vi "Post-Install Custom Action.vi"(10 "Variant":variant) -> (0 "error out":errorcluster)   [LabVIEW 2021]
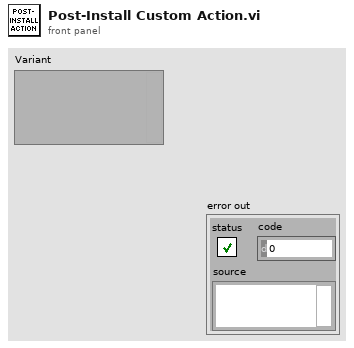
[diagram p1: front panel]
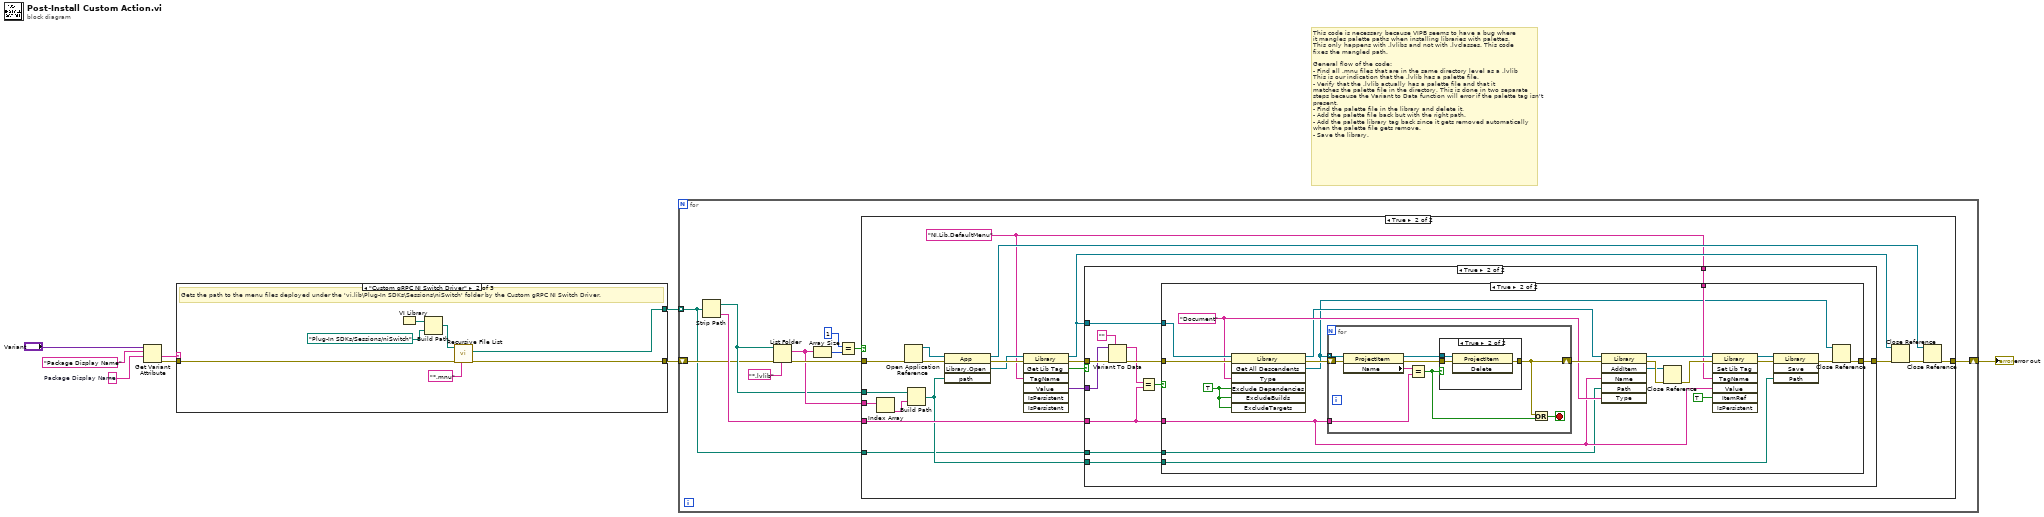
[diagram p0: block diagram]
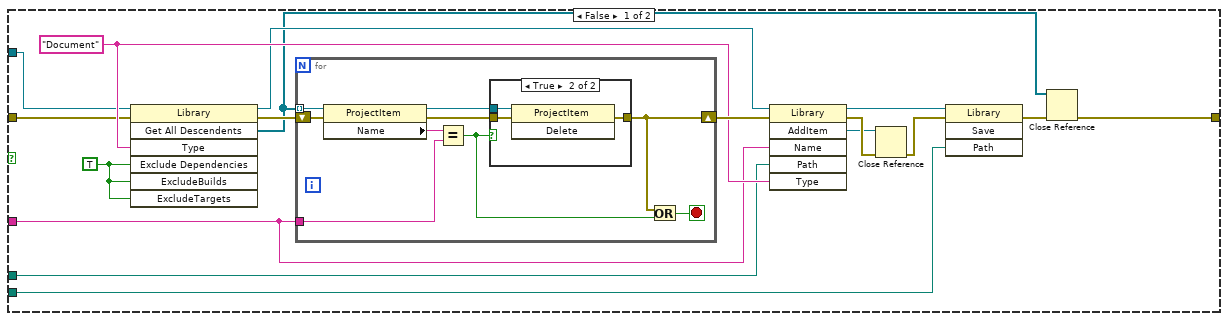
[diagram p4: hidden frame]
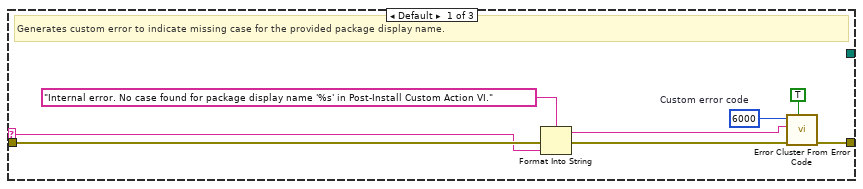
[diagram p7: hidden frame]
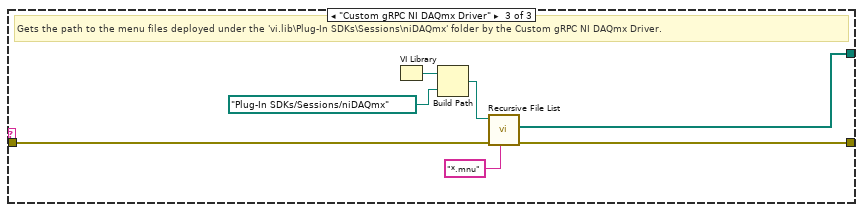
[diagram p8: hidden frame]
diagram:
  w7 = ""  # Package Display Name
  # "This code is necessary because VIPB seems to have a bug where\nit mangles palette paths when installing libraries with palettes.\nThis only happens with .lvlibs and not with .lvclasses. This code\nfixes the mangled path.\n\nGeneral flow of the code:\n- Find all .mnu files that are in the same directory level as a .lvlib\nThis is our indication that the .lvlib has a palette file.\n- Verify that the .lvlib actually has a palette file and that it\nmatches the palette file in the directory. This is done in two separate\nsteps because the Variant to Data function will error if the palette tag isn't\npresent.\n- Find the palette file in the library and delete it.\n- Add the palette file back but with the right path.\n- Add the palette library tag back since it gets removed automatically\nwhen the palette file gets remove.\n- Save the library."
  n1 = Get Variant Attribute(Variant="Variant", name="Package Display Name", default value (empty Variant)=w7) -> (value=w2:string, error out=w1:errorcluster)  [unwired: 1 in, 2 out]
  n2 = case shown="\"Custom gRPC NI Switch Driver\"" w2 {
    selector: w2 -> [w13 _ _]
    tunnel: [_ w19 w24] -> w3
    tunnel: [w16 w20 w25] -> w4
    tunnel: w1 -> [w14 w18 w26]
    frame Default {
      w11 = 6000  # Custom error code
      # "Generates custom error to indicate missing case for the provided package display name."
      n3 = Format Into String(format string="Internal error. No case found for package display name '%s' in Post-Install Custom Action VI.", error in=w14, w13) -> (resulting string=w12:string, error out=w15:errorcluster)  [unwired: 1 in]
      n4 = call <vilib>:"Error Cluster From Error Code.vi"("show call chain? (False)"=TRUE, "error in (no error)"=w15, "error message (\"\")"=w12, "error code (0)"=w11) -> ("error out"=w16:errorcluster)  [unwired: 5 in]
    }
    frame "Custom gRPC NI Switch Driver" {
      # "Gets the path to the menu files deployed under the 'vi.lib\\Plug-In SDKs\\Sessions\\niSwitch' folder by the Custom gRPC NI Switch Driver."
      n5 = VI Library() -> (path=w22:path)
      n6 = Build Path(base path=w22, name or relative path=path "Plug-In SDKs/Sessions/niSwitch") -> (appended path=w23:path)
      n7 = call <vilib>:"Recursive File List.vi"("pattern"="*.mnu", "error in (no error)"=w18, "Folder Path"=w23) -> ("error out"=w20:errorcluster, "All Files in Dir"=w19:path[])  [unwired: 4 in, 3 out]
    }
    frame "Custom gRPC NI DAQmx Driver" {
      # "Gets the path to the menu files deployed under the 'vi.lib\\Plug-In SDKs\\Sessions\\niDAQmx' folder by the Custom gRPC NI DAQmx Driver."
      n8 = VI Library() -> (path=w29:path)
      n9 = Build Path(base path=w29, name or relative path=path "Plug-In SDKs/Sessions/niDAQmx") -> (appended path=w30:path)
      n10 = call <vilib>:"Recursive File List.vi"("pattern"="*.mnu", "error in (no error)"=w26, "Folder Path"=w30) -> ("error out"=w25:errorcluster, "All Files in Dir"=w24:path[])  [unwired: 4 in, 3 out]
    }
  }
  n11 = for {
    shift-right: [w33] -> w6
    shift-left: w4 -> [w32]
    tunnel: w3 -> [w31] mode=indexing
    n12 = Strip Path(path=w31) -> (stripped path=w35:path, name=w39:string)
    n13 = List Folder(path=w35, pattern="*.lvlib", error in=w32) -> (filenames=w37:string[], error out=w38:errorcluster)  [unwired: 1 in, 2 out]
    n14 = Array Size(array=w37) -> (size(s)=w41:i32)
    n15 = Equal?(x=1, y=w41) -> (x = y?=w40:bool)
    n16 = case shown="True" w40 {
      tunnel: w38 -> [w42 w59]
      tunnel: w37 -> [_ w62]
      tunnel: w39 -> [_ w54]
      tunnel: w35 -> [_ w50]
      tunnel: [w42 w44] -> w33
      tunnel: w31 -> [_ w43]
      frame False {
      }
      frame True {
        w46 = "NI.Lib.DefaultMenu" ("Tag Name")
        n17 = Index Array(array=w62) -> (element=w49:string)  [unwired: 1 in]
        n18 = Open Application Reference(8:w59) -> (0:w61:errorcluster, 3:w60:refnum<vi>)  [unwired: 3 in]
        n19 = Build Path(base path=w50, name or relative path=w49) -> (appended path=w48:path)
        n20 = invoke class="App" method="Library.Open"(reference=w60, error in=w61, "path"=w48) -> (reference out=w51:refnum<vi>, error out=w58:errorcluster, "Open Library"=w55:refnum<vi>)  [unwired: 1 in, 1 out]
        n21 = invoke class="Library" method="Get Lib Tag"(reference=w55, error in=w58, "TagName"=w46) -> (reference out=w52:refnum<vi>, error out=w56:errorcluster, "GetTag"=w47:bool, "Value"=w57:variant)  [unwired: 4 in, 3 out]
        n22 = case shown="True" w47 {
          tunnel: w57 -> [_ w71]
          tunnel: w56 -> [w63 w72]
          tunnel: [w63 w75] -> w53
          tunnel: w52 -> [_ w74]
          tunnel: w48 -> [_ w73]
          tunnel: w54 -> [_ w67]
          tunnel: w46 -> [_ w65]
          tunnel: w43 -> [_ w64]
          frame False {
          }
          frame True {
            n23 = Variant To Data(error in=w72, type="", Variant=w71) -> (data=w68:string, error out=w70:errorcluster)
            n24 = Equal?(x=w68, y=w67) -> (x = y?=w66:bool)
            n25 = case shown="True" w66 {
              tunnel: [w76 w115] -> w75
              tunnel: w74 -> [w80 w126]
              tunnel: w73 -> [w77 w121]
              tunnel: w70 -> [w81 w120]
              tunnel: w67 -> [w79 w107]
              tunnel: w65 -> [_ w112]
              tunnel: w64 -> [w78 w106]
              frame False {
                w86 = "Document" ("Type")
                w84 = TRUE ("ExcludeDependencies")
                n26 = invoke class="Library" method="Get All Descendents"(reference=w80, error in=w81, "Type"=w86, "Exclude Dependencies"=w84, "ExcludeBuilds"=w84, "ExcludeTargets"=w84) -> (reference out=w83:refnum<vi>, error out=w92:errorcluster, "All Descendents"=w82:refnum<vi>[])  [unwired: 1 in, 4 out]
                n27 = for {
                  tunnel: w82 -> [w101] mode=indexing
                  shift-right: [w95] -> w91
                  shift-left: w92 -> [w97]
                  tunnel: w79 -> [w96]
                  stop <- w93 stop-if-true
                  n28 = property class="ProjectItem"(reference=w101, error in=w97) -> (reference out=w99:refnum<vi>, error out=w98:errorcluster, "Name"=w100:string)
                  n29 = Equal?(x=w100, y=w96) -> (x = y?=w94:bool)
                  n30 = case shown="True" w94 {
                    tunnel: w99 -> [_ w105]
                    tunnel: w98 -> [w102 w103]
                    tunnel: [w102 w104] -> w95
                    frame False {
                    }
                    frame True {
                      n31 = invoke class="ProjectItem" method="Delete"(reference=w105, error in=w103) -> (error out=w104:errorcluster)  [unwired: 1 in, 2 out]
                    }
                  }
                  n32 = Or(x=w95, y=w94) -> (x .or. y?=w93:bool)
                }
                n33 = invoke class="Library" method="AddItem"(reference=w83, error in=w91, "Name"=w79, "Path"=w78, "Type"=w86) -> (reference out=w85:refnum<vi>, error out=w89:errorcluster, "AddItem"=w88:refnum<vi>)  [unwired: 1 in, 3 out]
                n34 = Close Reference(reference=w88, error in (no error)=w89) -> (error out=w87:errorcluster)
                n35 = invoke class="Library" method="Save"(reference=w85, error in=w87, "Path"=w77) -> (error out=w90:errorcluster)  [unwired: 1 in, 3 out]
                n36 = Close Reference(reference=w82, error in (no error)=w90) -> (error out=w76:errorcluster)
              }
              frame True {
                w114 = "Document" ("Type")
                w110 = TRUE ("ExcludeDependencies")
                n37 = invoke class="Library" method="Get All Descendents"(reference=w126, error in=w120, "Type"=w114, "Exclude Dependencies"=w110, "ExcludeBuilds"=w110, "ExcludeTargets"=w110) -> (reference out=w109:refnum<vi>, error out=w125:errorcluster, "All Descendents"=w108:refnum<vi>[])  [unwired: 1 in, 4 out]
                n38 = for {
                  tunnel: w108 -> [w135] mode=indexing
                  shift-right: [w129] -> w124
                  shift-left: w125 -> [w131]
                  tunnel: w107 -> [w130]
                  stop <- w127 stop-if-true
                  n39 = property class="ProjectItem"(reference=w135, error in=w131) -> (reference out=w133:refnum<vi>, error out=w132:errorcluster, "Name"=w134:string)
                  n40 = Equal?(x=w134, y=w130) -> (x = y?=w128:bool)
                  n41 = case shown="True" w128 {
                    tunnel: w133 -> [_ w139]
                    tunnel: w132 -> [w136 w137]
                    tunnel: [w136 w138] -> w129
                    frame False {
                    }
                    frame True {
                      n42 = invoke class="ProjectItem" method="Delete"(reference=w139, error in=w137) -> (error out=w138:errorcluster)  [unwired: 1 in, 2 out]
                    }
                  }
                  n43 = Or(x=w129, y=w128) -> (x .or. y?=w127:bool)
                }
                n44 = invoke class="Library" method="AddItem"(reference=w109, error in=w124, "Name"=w107, "Path"=w106, "Type"=w114) -> (reference out=w113:refnum<vi>, error out=w118:errorcluster, "AddItem"=w117:refnum<vi>)  [unwired: 1 in, 3 out]
                n45 = Close Reference(reference=w117, error in (no error)=w118) -> (error out=w116:errorcluster)
                n46 = invoke class="Library" method="Set Lib Tag"(reference=w113, error in=w116, "TagName"=w112, "Value"=w107, "ItemRef"=TRUE ("Is Persistent")) -> (reference out=w123:refnum<vi>, error out=w122:errorcluster)  [unwired: 2 in, 5 out]
                n47 = invoke class="Library" method="Save"(reference=w123, error in=w122, "Path"=w121) -> (error out=w119:errorcluster)  [unwired: 1 in, 3 out]
                n48 = Close Reference(reference=w108, error in (no error)=w119) -> (error out=w115:errorcluster)
              }
            }
          }
        }
        n49 = Close Reference(reference=w52, error in (no error)=w53) -> (error out=w45:errorcluster)
        n50 = Close Reference(reference=w51, error in (no error)=w45) -> (error out=w44:errorcluster)
      }
    }
  }
  "error out" <- w6
